vi "C_CIF_Encode_RT.vi"(8 "error in (no error)":errorcluster, 9 "little endian":bool, 10 "pcap":u8[](array[numeric]), 11 "tx in":u8[](array[numeric])) -> (0 "error out":errorcluster, 1 "result":T1, 3 "tx out":u8[](array[numeric]))   [LabVIEW 2021, in "CANsub_C.lvlib"]
doc: "Converts pcap CAN packets (NI CIF format) to WebSocket frames for one TCP Write, in the tx buffer of the caller. Remote frames and error frames are not converted and are counted in n rejected. The tx buffer must hold 174 bytes for each packet. If consumed is less than the size of pcap, the remaining bytes were not converted. Loop-safe: no allocation, bounded time."
uses:
  CANsub_C.lvlib
  C_CIF_Encode_Result.ctl
  codec_vis/CANsub_Codec.lvlib
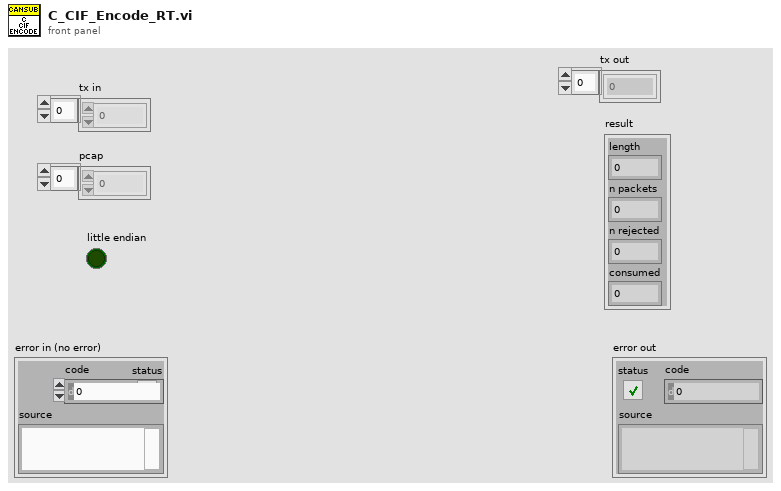
[diagram p1: front panel]
types:
  T1 = typedef "CANsub_C.lvlib/C_CIF_Encode_Result.ctl" = cluster{"length":i32, "n packets":i32, "n rejected":i32, "consumed":i32}
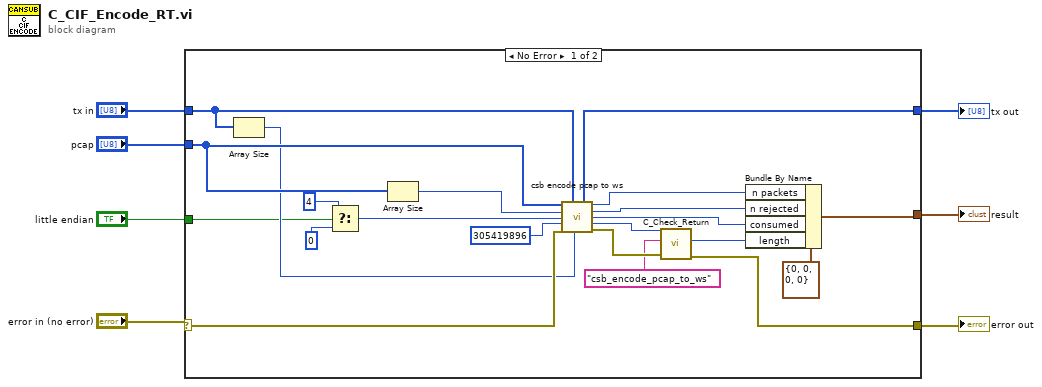
[diagram p0: block diagram]
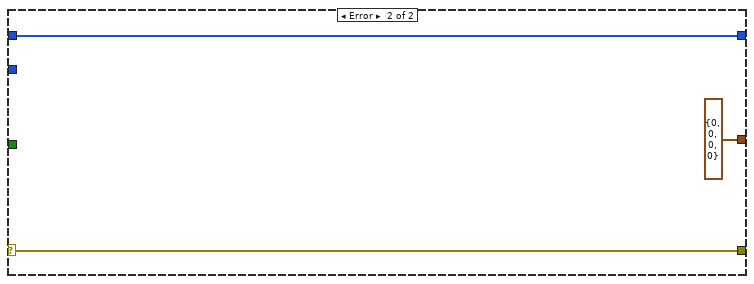
[diagram p2: hidden frame]
diagram:
  n1 = case shown="No Error" "error in (no error)" {
    selector: "error in (no error)" -> [w22 w30]
    tunnel: [w10 w31] -> w6
    tunnel: "tx in" -> [w21 w31]
    tunnel: [w8 w30] -> w4
    tunnel: [w9 T1 {"length"=0, "n packets"=0, "n rejected"=0, "consumed"=0} ("result")] -> w3
    tunnel: "pcap" -> [w26 _]
    tunnel: "little endian" -> [w19 _]
    frame No Error {
      n2 = Array Size(array=w21) -> (size(s)=w20:i32)
      n3 = Select(t=4, s=w19, f=0) -> (s? t:f=w24:i32)
      n4 = Array Size(array=w26) -> (size(s)=w25:i32)
      n5 = call "csb encode pcap to ws.vi"("in"=w26, "out"=w21, "in_len"=w25, "options"=w24, "mask"=u32 305419896, "error in (no error)"=w22, "out_cap"=w20) -> ("out out"=w10:u8[], "n_packets"=w13:i32, "n_rejected"=w12:i32, "consumed"=w11:i32, "function return"=w18:i32, "error out"=w17:errorcluster)  [unwired: 3 in]
      n6 = call "C_Check_Return.vi"("error in (no error)"=w17, "function name"="csb_encode_pcap_to_ws", "function return"=w18) -> ("error out"=w8:errorcluster, "length"=w14:i32)  [unwired: 6 in, 1 out]
      n7 = Bundle By Name(cluster=T1 {"length"=0, "n packets"=0, "n rejected"=0, "consumed"=0} ("C_CIF_Encode_Result"), "n packets"=w13, "n rejected"=w12, "consumed"=w11, "length"=w14) -> (w9:T1)
    }
    frame Error {
    }
  }
  "result" <- w3
  "error out" <- w4
  "tx out" <- w6
